vi "fix.vi"(8 "error in (no error)":errorcluster, 10 "result":refnum<class "VideoFile.lvclass">, 11 "AudioMixer in":refnum<class "AudioMixer.lvclass">) -> (0 "error out":errorcluster, 2 "result out":refnum<class "VideoFile.lvclass">, 3 "AudioMixer out":refnum<class "AudioMixer.lvclass">)   [LabVIEW 2018, in "AudioMixer.lvclass"]
uses:
  AudioMixer.lvclass
  VideoFile Class/VideoFile.lvclass
  ConsoleOut/Print Options.ctl
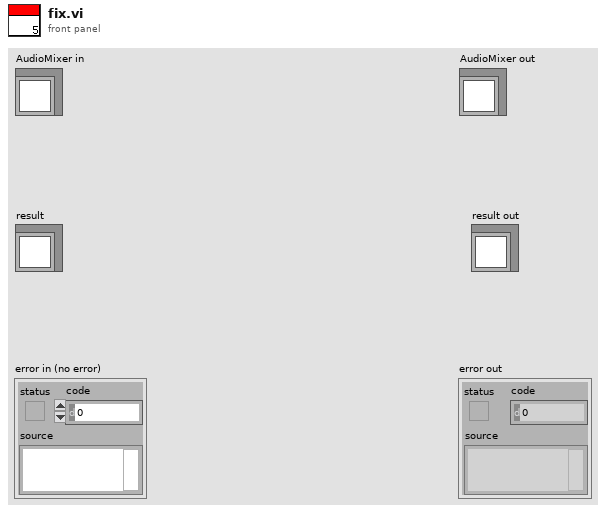
[diagram p1: front panel]
types:
  T1 = typedef "Print Options.ctl" = enum16{"Create", "Get Reference", "Print", "Print Header", "Close"}
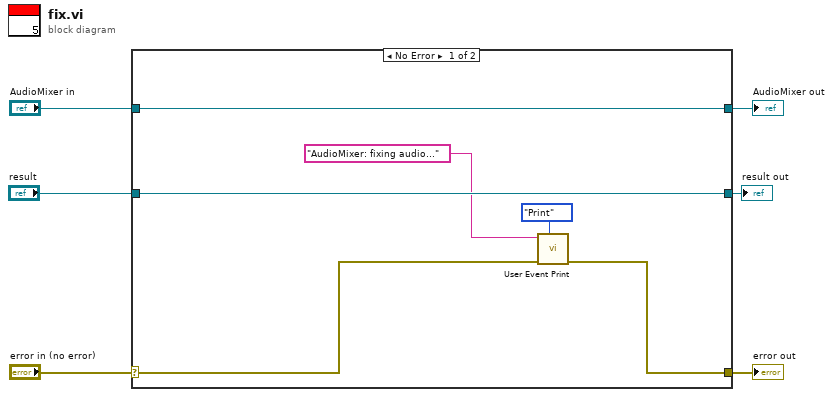
[diagram p0: block diagram]
diagram:
  n1 = case shown="No Error" "error in (no error)" {
    selector: "error in (no error)" -> [w11 w15]
    tunnel: [w9 w15] -> w5
    tunnel: [w12 w14] -> w3
    tunnel: "AudioMixer in" -> [w12 w14]
    tunnel: "result" -> [w10 w13]
    tunnel: [w10 w13] -> w1
    frame No Error {
      n2 = call "User Event Print.vi"("Options"=Print_Options."Print", "error in (no error)"=w11, "String to Print"="AudioMixer: fixing audio..." ("message")) -> ("error out"=w9:errorcluster)  [unwired: 7 in, 1 out]
    }
    frame Error {
    }
  }
  "error out" <- w5
  "AudioMixer out" <- w3
  "result out" <- w1
